vi "CANsub_REST_Status.vi"(8 "error in (no error)":errorcluster, 9 "channel":u8, 10 "host":string, 11 "client handle":T1) -> (0 "error out":errorcluster, 2 "device status":T2, 3 "client handle out":T1)   [LabVIEW 2021, in "CANsub_Common.lvlib"]
doc: "Reads the status of one CAN channel from the device (GET /api/can/): state, frame counters, bus load and error counters. Opens and closes one HTTPS connection for each call. Setup/teardown only: do not call in a periodic loop (allocates).\n\nTime limit 500 ms, so that a server that does not answer blocks the caller for 0.5 s at most."
uses:
  CANsub_Common.lvlib
  Typedefs/HTTP_Method.ctl
  Typedefs/CANsub_Device_Status.ctl
  <vilib>/httpClient/ClientHandle.ctl
  <vilib>/httpClient/LabVIEWHTTPClient.lvlib
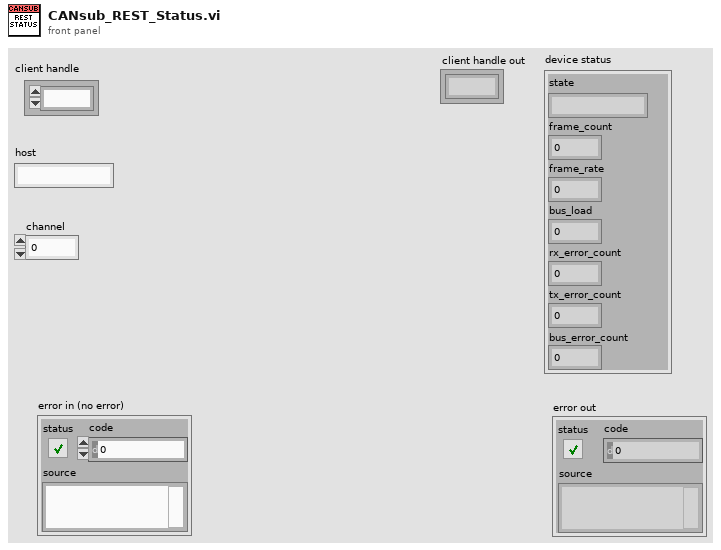
[diagram p1: front panel]
types:
  T1 = typedef "LabVIEWHTTPClient.lvlib/ClientHandle.ctl" = refnum<k1>
  T2 = typedef "CANsub_Common.lvlib/CANsub_Device_Status.ctl" = cluster{"state":string, "frame_count":u32, "frame_rate":dbl, "bus_load":dbl, "rx_error_count":u32, "tx_error_count":u32, "bus_error_count":u32}
  T3 = typedef "CANsub_Common.lvlib/HTTP_Method.ctl" = enum16{"GET", "PUT", "POST", "DELETE"}
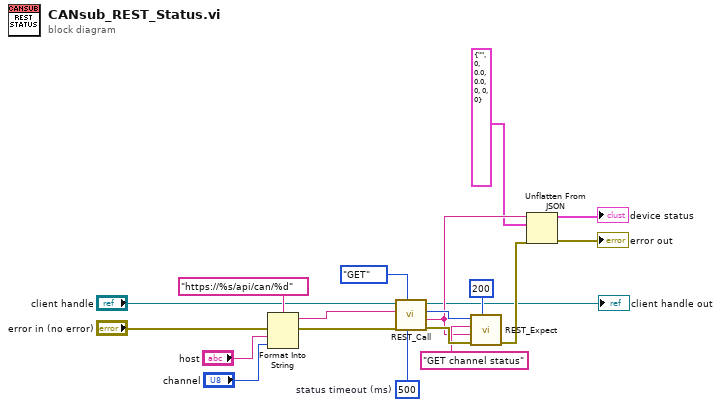
[diagram p0: block diagram]
diagram:
  w1 = 500  # status timeout (ms)
  n1 = Format Into String(format string="https://%s/api/can/%d", error in="error in (no error)", "host", "channel") -> (resulting string=w10:string, error out=w11:errorcluster)  [unwired: 1 in]
  n2 = call "REST_Call.vi"("timeout ms (5000)"=w1, "method"=HTTP_Method."GET", "error in (no error)"=w11, "url"=w10, "client handle"="client handle") -> ("error out"=w18:errorcluster, "response"=w9:string, "status"=w16:i32, "client handle out"=→"client handle out":T1)  [unwired: 3 in]
  n3 = call "REST_Expect.vi"("expected"=200, "error in (no error)"=w18, "response"=w9, "what"="GET channel status", "status"=w16) -> ("error out"=w7:errorcluster)  [unwired: 5 in, 1 out]
  n4 = Unflatten From JSON(JSON string=w9, type and defaults=T2 {"state"="", "frame_count"=0, "frame_rate"=0.0, "bus_load"=0.0, "rx_error_count"=0, "tx_error_count"=0, "bus_error_count"=0} ("CANsub_Device_Status"), error in (no error)=w7) -> (value=→"device status":T2, error out=→"error out":errorcluster)  [unwired: 4 in]
